vi "Index Tags.vi"(4 "Don't Create":bool, 6 "Tag Type":T1, 8 "error in (no error)":errorcluster, 9 "Tag":string, 10 "Group Index":i32, 11 "bt_Blackboard in":refnum<class "Blackboard.lvclass">) -> (0 "error out":errorcluster, 1 "New Tag?":bool, 2 "Value":refnum<class "Abs_Value.lvclass">, 3 "bt_Blackboard out":refnum<class "Blackboard.lvclass">)   [LabVIEW 2021, in "Blackboard.lvclass"]
uses:
  Blackboard.lvclass
  <vilib>/Utility/Data Type/Type Definitions/Data Type.ctl
  <vilib>/TSA/Abstract Data Classes/Abs_Types/Value/Abs_Value.lvclass
  Blackboard.lvclass/Blackboard.ctl
  <vilib>/TSA/Omni-Bus/Local Bus/Support/DBL/Local Bus_DBL.lvclass
  C:/Program Files (x86)/National Instruments/LabVIEW 2021/vi.lib/TSA/Abstract Data Classes/Abs_Types/Value/Abs_Value.lvclass
  <vilib>/TSA/Omni-Bus/Local Bus/Support/SGL/Local Bus_SGL.lvclass
  <vilib>/TSA/Omni-Bus/Local Bus/Support/EXT/Local Bus_EXT.lvclass
  <vilib>/TSA/Omni-Bus/Local Bus/Support/Bool/Local Bus_Boolean.lvclass
  <vilib>/TSA/Omni-Bus/Local Bus/Support/STR/Local Bus_String.lvclass
  <vilib>/TSA/Omni-Bus/Local Bus/Support/Variant/Local Bus_Variant.lvclass
  <vilib>/TSA/Omni-Bus/Local Bus/Support/WFM/Local Bus_Waveform.lvclass
  <vilib>/TSA/Omni-Bus/Local Bus/Support/Time/Local Bus_Time.lvclass
  <vilib>/TSA/Omni-Bus/Local Bus/Support/U8/Local Bus_U8.lvclass
  <vilib>/TSA/Omni-Bus/Local Bus/Support/U16/Local Bus_U16.lvclass
  <vilib>/TSA/Omni-Bus/Local Bus/Support/U32/Local Bus_U32.lvclass
  <vilib>/TSA/Omni-Bus/Local Bus/Support/U64/Local Bus_U64.lvclass
  <vilib>/TSA/Omni-Bus/Local Bus/Support/I8/Local Bus_I8.lvclass
  <vilib>/TSA/Omni-Bus/Local Bus/Support/I16/Local Bus_I16.lvclass
  <vilib>/TSA/Omni-Bus/Local Bus/Support/I32/Local Bus_I32.lvclass
  <vilib>/TSA/Omni-Bus/Local Bus/Support/I64/Local Bus_I64.lvclass
  <vilib>/TSA/Omni-Bus/Local Bus/Support/CSGL/Local Bus_CSGL.lvclass
  <vilib>/TSA/Omni-Bus/Local Bus/Support/CDBL/Local Bus_CDBL.lvclass
  <vilib>/TSA/Omni-Bus/Local Bus/Support/CEXT/Local Bus_CEXT.lvclass
  <vilib>/TSA/Omni-Bus/Local Bus/Support/Type/Local Bus_Type.lvclass
  <vilib>/TSA/Abstract Data Classes/Abs_Types/Type/Abs_Type.lvclass
  C:/Program Files (x86)/National Instruments/LabVIEW 2021/vi.lib/TSA/Abstract Data Classes/Abs_Types/Type/Abs_Type.lvclass
  C:/Program Files (x86)/National Instruments/LabVIEW 2021/vi.lib/TSA/Abstract Data Classes/Abs_Types/Double Float/Abs_Double Float.lvclass
  C:/Program Files (x86)/National Instruments/LabVIEW 2021/vi.lib/TSA/Abstract Data Classes/Abs_Types/Floating Point/Abs_Floating Point.lvclass
  C:/Program Files (x86)/National Instruments/LabVIEW 2021/vi.lib/TSA/Abstract Data Classes/Abs_Types/Numeric/Abs_Numeric.lvclass
  C:/Program Files (x86)/National Instruments/LabVIEW 2021/vi.lib/TSA/Omni-Bus/Local Bus/Support/DBL/Local Bus_DBL.lvclass
  C:/Program Files (x86)/National Instruments/LabVIEW 2021/vi.lib/TSA/Omni-Bus/Local Bus/Support/Interface/Local Bus_Int.lvclass
  C:/Program Files (x86)/National Instruments/LabVIEW 2021/vi.lib/TSA/Abstract Data Classes/Abs_Types/Single Float/Abs_Single Float.lvclass
  C:/Program Files (x86)/National Instruments/LabVIEW 2021/vi.lib/TSA/Omni-Bus/Local Bus/Support/SGL/Local Bus_SGL.lvclass
  C:/Program Files (x86)/National Instruments/LabVIEW 2021/vi.lib/TSA/Abstract Data Classes/Abs_Types/Extended Float/Abs_Extended Float.lvclass
  C:/Program Files (x86)/National Instruments/LabVIEW 2021/vi.lib/TSA/Omni-Bus/Local Bus/Support/EXT/Local Bus_EXT.lvclass
  C:/Program Files (x86)/National Instruments/LabVIEW 2021/vi.lib/TSA/Abstract Data Classes/Abs_Types/Boolean/Abs_Boolean.lvclass
  C:/Program Files (x86)/National Instruments/LabVIEW 2021/vi.lib/TSA/Omni-Bus/Local Bus/Support/Bool/Local Bus_Boolean.lvclass
  C:/Program Files (x86)/National Instruments/LabVIEW 2021/vi.lib/TSA/Abstract Data Classes/Abs_Types/String/Abs_String.lvclass
  C:/Program Files (x86)/National Instruments/LabVIEW 2021/vi.lib/TSA/Omni-Bus/Local Bus/Support/STR/Local Bus_String.lvclass
  C:/Program Files (x86)/National Instruments/LabVIEW 2021/vi.lib/TSA/Abstract Data Classes/Abs_Types/Variant/Abs_Variant.lvclass
  C:/Program Files (x86)/National Instruments/LabVIEW 2021/vi.lib/TSA/Omni-Bus/Local Bus/Support/Variant/Local Bus_Variant.lvclass
  C:/Program Files (x86)/National Instruments/LabVIEW 2021/vi.lib/TSA/Abstract Data Classes/Abs_Types/Waveform/Abs_Waveform.lvclass
  C:/Program Files (x86)/National Instruments/LabVIEW 2021/vi.lib/TSA/Abstract Data Classes/Abs_Types/Collections/Vectors/Vector/Vector.lvclass
  C:/Program Files (x86)/National Instruments/LabVIEW 2021/vi.lib/TSA/Abstract Data Classes/Abs_Types/Iterator/Iterator.lvclass
  C:/Program Files (x86)/National Instruments/LabVIEW 2021/vi.lib/TSA/Abstract Data Classes/Abs_Types/Collections/Vectors/Vector_DBL/Vector_DBL.lvclass
  C:/Program Files (x86)/National Instruments/LabVIEW 2021/vi.lib/TSA/Omni-Bus/Local Bus/Support/WFM/Local Bus_Waveform.lvclass
  C:/Program Files (x86)/National Instruments/LabVIEW 2021/vi.lib/TSA/Abstract Data Classes/Abs_Types/Time/Abs_Time.lvclass
  C:/Program Files (x86)/National Instruments/LabVIEW 2021/vi.lib/TSA/Omni-Bus/Local Bus/Support/Time/Local Bus_Time.lvclass
  C:/Program Files (x86)/National Instruments/LabVIEW 2021/vi.lib/TSA/Abstract Data Classes/Abs_Types/U8 Integer/Abs_U8 Integer.lvclass
  C:/Program Files (x86)/National Instruments/LabVIEW 2021/vi.lib/TSA/Abstract Data Classes/Abs_Types/Integer/Abs_Integer.lvclass
  C:/Program Files (x86)/National Instruments/LabVIEW 2021/vi.lib/TSA/Omni-Bus/Local Bus/Support/U8/Local Bus_U8.lvclass
  C:/Program Files (x86)/National Instruments/LabVIEW 2021/vi.lib/TSA/Abstract Data Classes/Abs_Types/U16 Integer/Abs_U16 Integer.lvclass
  C:/Program Files (x86)/National Instruments/LabVIEW 2021/vi.lib/TSA/Omni-Bus/Local Bus/Support/U16/Local Bus_U16.lvclass
  C:/Program Files (x86)/National Instruments/LabVIEW 2021/vi.lib/TSA/Abstract Data Classes/Abs_Types/U32 Integer/Abs_U32 Integer.lvclass
  C:/Program Files (x86)/National Instruments/LabVIEW 2021/vi.lib/TSA/Omni-Bus/Local Bus/Support/U32/Local Bus_U32.lvclass
  C:/Program Files (x86)/National Instruments/LabVIEW 2021/vi.lib/TSA/Abstract Data Classes/Abs_Types/U64 Integer/Abs_U64 Integer.lvclass
  C:/Program Files (x86)/National Instruments/LabVIEW 2021/vi.lib/TSA/Omni-Bus/Local Bus/Support/U64/Local Bus_U64.lvclass
  C:/Program Files (x86)/National Instruments/LabVIEW 2021/vi.lib/TSA/Abstract Data Classes/Abs_Types/I8 Integer/Abs_I8 Integer.lvclass
  C:/Program Files (x86)/National Instruments/LabVIEW 2021/vi.lib/TSA/Omni-Bus/Local Bus/Support/I8/Local Bus_I8.lvclass
  C:/Program Files (x86)/National Instruments/LabVIEW 2021/vi.lib/TSA/Abstract Data Classes/Abs_Types/I16 Integer/Abs_I16 Integer.lvclass
  C:/Program Files (x86)/National Instruments/LabVIEW 2021/vi.lib/TSA/Omni-Bus/Local Bus/Support/I16/Local Bus_I16.lvclass
  C:/Program Files (x86)/National Instruments/LabVIEW 2021/vi.lib/TSA/Abstract Data Classes/Abs_Types/I32 Integer/Abs_I32 Integer.lvclass
  C:/Program Files (x86)/National Instruments/LabVIEW 2021/vi.lib/TSA/Omni-Bus/Local Bus/Support/I32/Local Bus_I32.lvclass
  C:/Program Files (x86)/National Instruments/LabVIEW 2021/vi.lib/TSA/Abstract Data Classes/Abs_Types/I64 Integer/Abs_I64 Integer.lvclass
  C:/Program Files (x86)/National Instruments/LabVIEW 2021/vi.lib/TSA/Omni-Bus/Local Bus/Support/I64/Local Bus_I64.lvclass
  C:/Program Files (x86)/National Instruments/LabVIEW 2021/vi.lib/TSA/Abstract Data Classes/Abs_Types/Complex Single Float/Abs_Complex Single Float.lvclass
  C:/Program Files (x86)/National Instruments/LabVIEW 2021/vi.lib/TSA/Omni-Bus/Local Bus/Support/CSGL/Local Bus_CSGL.lvclass
  C:/Program Files (x86)/National Instruments/LabVIEW 2021/vi.lib/TSA/Abstract Data Classes/Abs_Types/Complex Double Float/Abs_Complex Double Float.lvclass
  C:/Program Files (x86)/National Instruments/LabVIEW 2021/vi.lib/TSA/Omni-Bus/Local Bus/Support/CDBL/Local Bus_CDBL.lvclass
  C:/Program Files (x86)/National Instruments/LabVIEW 2021/vi.lib/TSA/Abstract Data Classes/Abs_Types/Complex Extended Float/Abs_Complex Extended Float.lvclass
  C:/Program Files (x86)/National Instruments/LabVIEW 2021/vi.lib/TSA/Omni-Bus/Local Bus/Support/CEXT/Local Bus_CEXT.lvclass
  <vilib>/Utility/Data Type/NI_Data Type.lvlib
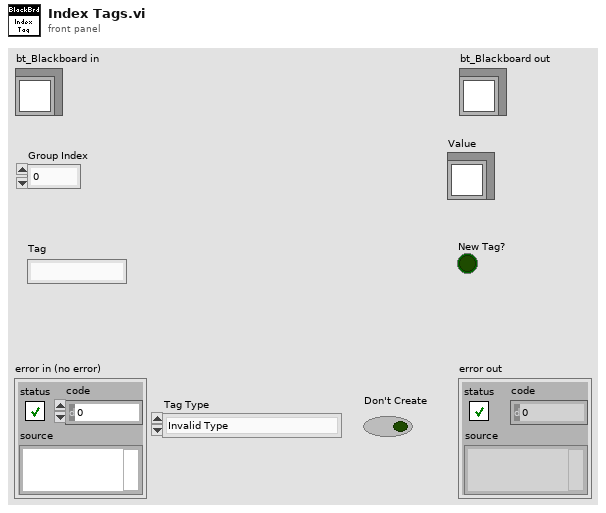
[diagram p1: front panel]
types:
  T1 = typedef "NI_Data Type.lvlib/Data Type.ctl" = enum8{"Invalid Type", "Void", "I8", "I16", "I32", "I64", "U8", "U16", "U32", "U64", "Single Float", "Double Float", "Extended Float", "Single Complex", "Double Complex", "Extended Complex", "Enum U8", "Enum U16", "Enum U32", "Enum U64", "Single Float With Unit", "Double Float With Unit", "Extended Float With Unit", "Single Complex with Unit", "Double Complex with Unit", "Extended Complex with Unit", "Boolean", "String", "Path", "Picture", "Tag", "Array", "Cluster", "Variant", "LV Variant", "Waveform", "Timestamp", "Digital Waveform", "Digital Data", "ExpressData", "Refnum", "External Data", "VI", "Poly VI", "LabVIEW Class Instance", "Fixed Point", "Set Collection", "Map Collection"}
  T2 = typedef "Blackboard.lvclass/Groups Type.ctl" = cluster{"Data":T3[], "Map":T6}
  T3 = typedef "Blackboard.lvclass/Data DVR Type.ctl" = cluster{"Tags":T4, "Data Refs":T5}
  T4 = typedef "Blackboard.lvclass/Tags Map Type.ctl" = map{string, refnum<class "Abs_Value.lvclass">}
  T5 = typedef "Local Bus.lvclass/Data Value References.ctl" = cluster{"Boolean":refnum<data-value>, "String":refnum<data-value>, "DBL":refnum<data-value>, "SGL":refnum<data-value>, "EXT":refnum<data-value>, "U8":refnum<data-value>, "U16":refnum<data-value>, "U32":refnum<data-value>, "U64":refnum<data-value>, "I8":refnum<data-value>, "I16":refnum<data-value>, "I32":refnum<data-value>, "I64":refnum<data-value>, "CDBL":refnum<data-value>, "CSGL":refnum<data-value>, "CEXT":refnum<data-value>, "Time":refnum<data-value>, "Variant":refnum<data-value>, "Waveform":refnum<data-value>, "Type":refnum<data-value>}
  T6 = typedef "Blackboard.lvclass/Group Map Type.ctl" = map{string, i32}
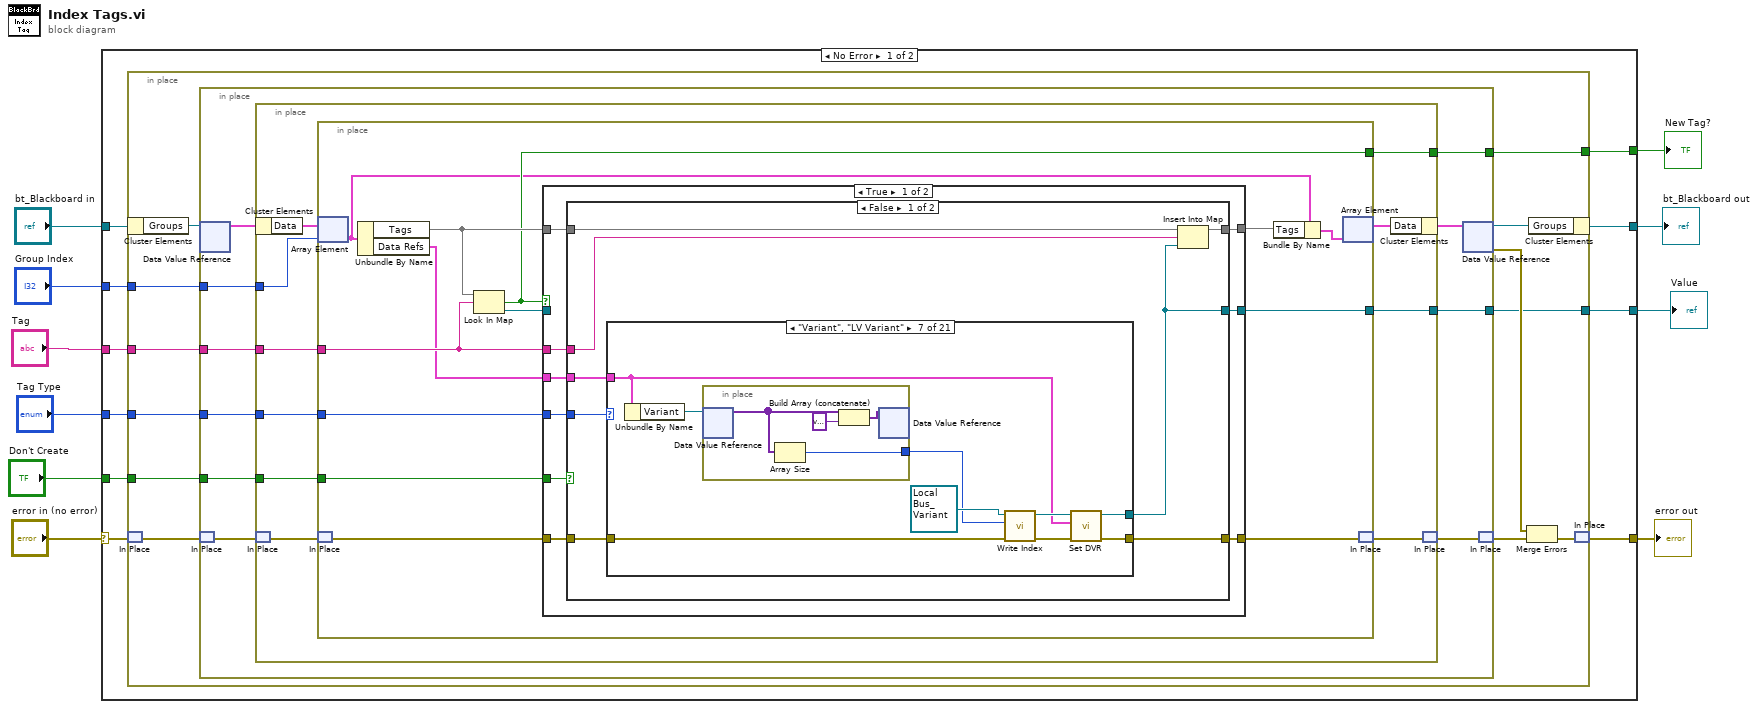
[diagram p0: block diagram]
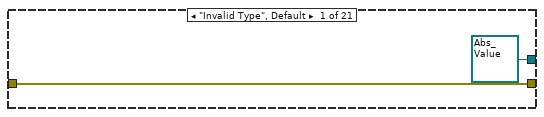
[diagram p2: hidden frame]
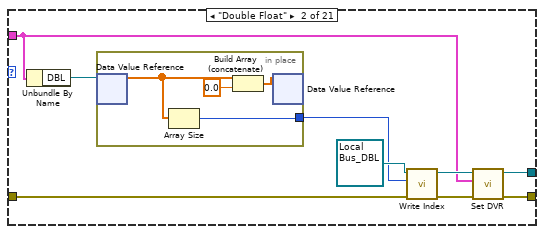
[diagram p3: hidden frame]
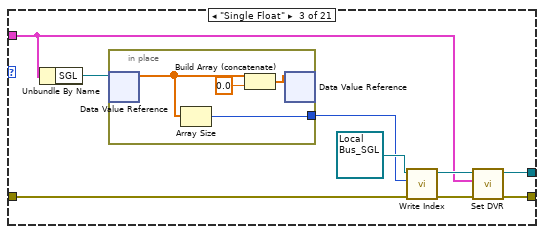
[diagram p4: hidden frame]
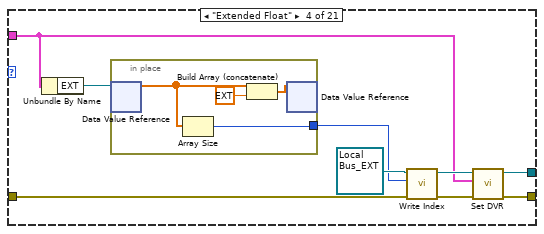
[diagram p5: hidden frame]
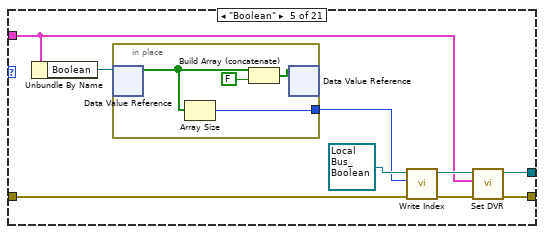
[diagram p6: hidden frame]
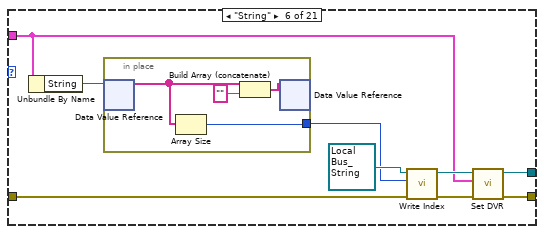
[diagram p7: hidden frame]
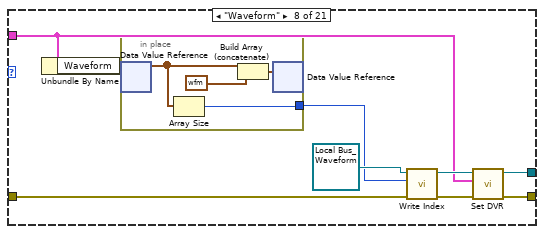
[diagram p8: hidden frame]
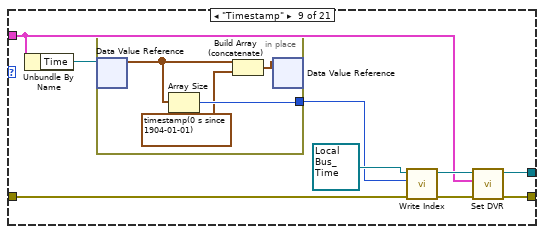
[diagram p9: hidden frame]
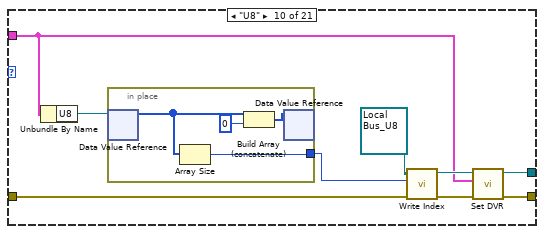
[diagram p10: hidden frame]
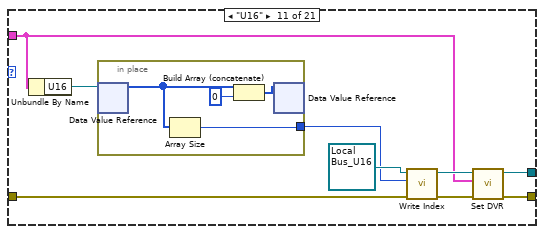
[diagram p11: hidden frame]
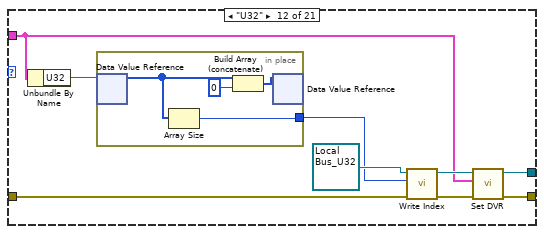
[diagram p12: hidden frame]
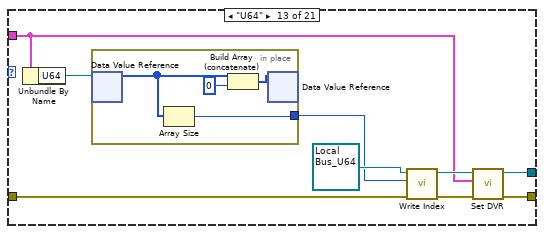
[diagram p13: hidden frame]
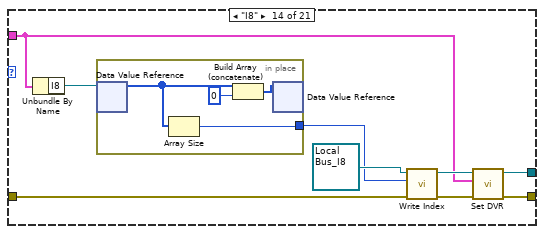
[diagram p14: hidden frame]
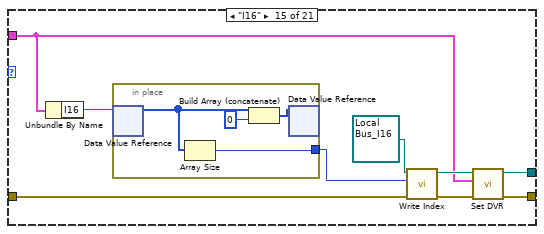
[diagram p15: hidden frame]
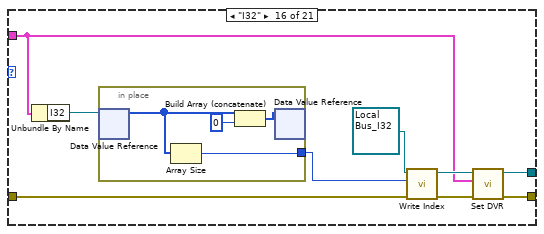
[diagram p16: hidden frame]
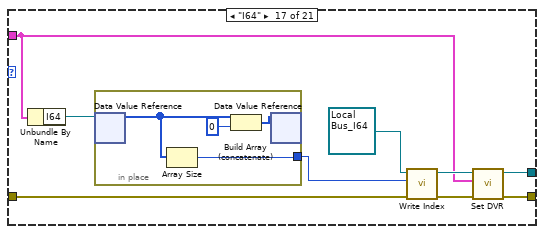
[diagram p17: hidden frame]
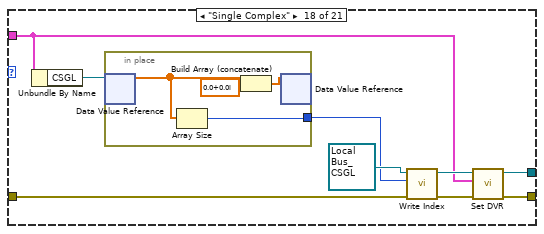
[diagram p18: hidden frame]
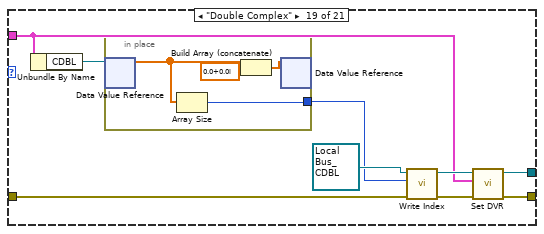
[diagram p19: hidden frame]
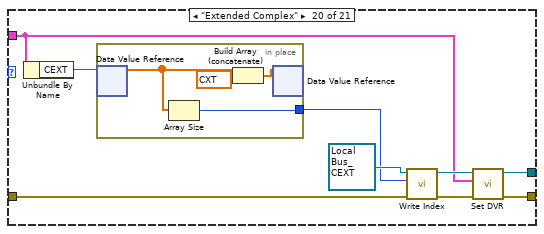
[diagram p20: hidden frame]
diagram:
  n1 = case shown="No Error" "error in (no error)" {
    selector: "error in (no error)" -> [w16 w355]
    tunnel: [w15 w355] -> w9
    tunnel: [w18 w354] -> w7
    tunnel: "bt_Blackboard in" -> [w19 w354]
    tunnel: "Tag" -> [w20 _]
    tunnel: "Group Index" -> [w17 _]
    tunnel: [w14 _] -> w4
    tunnel: [w13 _] -> w2
    tunnel: "Tag Type" -> [w12 _]
    tunnel: "Don't Create" -> [w11 _]
    frame No Error {
      n2 = in-place {
        in-place-border: w20 -> [w32]
        in-place-border: w17 -> [w31]
        in-place-border: [w30] -> w14
        in-place-border: [w23] -> w13
        in-place-border: w12 -> [w22]
        in-place-border: w11 -> [w21]
        n3 = in-place-cluster #1(w19) -> ("Groups"=w29:refnum<data-value>)
        n4 = in-place-match #2(w16) -> (w28:errorcluster)
        n5 = in-place {
          in-place-border: w32 -> [w42]
          in-place-border: w31 -> [w41]
          in-place-border: [w40] -> w30
          in-place-border: [w35] -> w23
          in-place-border: w22 -> [w34]
          in-place-border: w21 -> [w33]
          n6 = in-place-dvr #3(w29) -> (w39:T2)  [unwired: 1 out]
          n7 = in-place-match #4(w28) -> (w37:errorcluster)
          n8 = in-place {
            in-place-border: w42 -> [w52]
            in-place-border: w41 -> [w51]
            in-place-border: [w50] -> w40
            in-place-border: [w45] -> w35
            in-place-border: w34 -> [w44]
            in-place-border: w33 -> [w43]
            n9 = in-place-cluster #5(w39) -> ("Data"=w49:T3[])
            n10 = in-place-match #6(w37) -> (w47:errorcluster)
            n11 = in-place {
              in-place-border: w52 -> [w57]
              in-place-border: [w60] -> w50
              in-place-border: [w59] -> w45
              in-place-border: w44 -> [w55]
              in-place-border: w43 -> [w53]
              n12 = in-place-array #7(w49, w51) -> (w54:T3)
              n13 = in-place-match #8(w47) -> (w65:errorcluster)
              n14 = Unbundle By Name(w54) -> ("Tags"=w63:T4, "Data Refs"=w56:T5)
              n15 = Look In Map(map=w63, key=w57) -> (key not found?=w60:bool, value=w61:refnum<class "Abs_Value.lvclass">)  [unwired: 1 in]
              n16 = case shown="True" w60 {
                tunnel: w63 -> [w74 w353]
                tunnel: [w73 w353] -> w62
                tunnel: w65 -> [w70 w352]
                tunnel: [w69 w352] -> w64
                tunnel: w61 -> [_ w351]
                tunnel: [w67 w351] -> w59
                tunnel: w57 -> [w72 _]
                tunnel: w56 -> [w71 _]
                tunnel: w55 -> [w68 _]
                tunnel: w53 -> [w66 _]
                frame True {
                  n17 = case shown="False" w66 {
                    tunnel: w74 -> [w82 w350]
                    tunnel: [w81 w350] -> w73
                    tunnel: w72 -> [w80 _]
                    tunnel: w71 -> [w79 _]
                    tunnel: w70 -> [w78 w348]
                    tunnel: [w77 w348] -> w69
                    tunnel: w68 -> [w76 _]
                    tunnel: [w75 refnum<class "Abs_Value.lvclass"> refnum ("Local Bus_DBL out")] -> w67
                    frame False {
                      n18 = case shown="\"Variant\", \"LV Variant\"" w76 {
                        tunnel: [w84 w93 w106 w119 w132 w145 w158 w171 w184 w197 w210 w223 w236 w249 w262 w275 w288 w301 w314 w327 w336] -> w77
                        tunnel: w79 -> [_ w86 w99 w112 w125 w138 w151 w164 w177 w190 w203 w216 w229 w242 w255 w268 w281 w294 w307 w320 w339]
                        tunnel: [refnum<class "Abs_Value.lvclass"> refnum ("Local Bus_DBL out") w92 w105 w118 w131 w144 w157 w170 w183 w196 w209 w222 w235 w248 w261 w274 w287 w300 w313 w326 w332] -> w75
                        tunnel: w78 -> [w84 w91 w104 w117 w130 w143 w156 w169 w182 w195 w208 w221 w234 w247 w260 w273 w286 w299 w312 w325 w343]
                        frame "Invalid Type", Default {
                        }
                        frame "Double Float" {
                          n19 = Unbundle By Name(w86) -> ("DBL"=w87:refnum<data-value>)
                          n20 = in-place {
                            in-place-border: [w95] -> w85
                            n21 = in-place-dvr #9(w87) -> (w96:dbl[])  [unwired: 1 out]
                            n22 = Array Size(array=w96) -> (size(s)=w95:i32)
                            n23 = Build Array (concatenate)(w96, 0.0 ("element")) -> (w97:dbl[])
                            n24 = in-place-dvr #9(w97) -> ()  [unwired: 2 out]
                          }
                          n25 = call-dynamic "Write Index.vi"("error in (no error)"=w91, "Index"=w85, "Local Bus_Access in"=refnum<class "Local Bus_DBL.lvclass"> refnum ("Local Bus_DBL.lvclass")) -> ("error out"=w90:errorcluster, "Local Bus_Access out"=w89:refnum<class "Local Bus_DBL.lvclass">)  [unwired: 7 in]
                          n26 = call-dynamic "Set DVR.vi"("error in (no error)"=w90, "Type Counts"=w86, "Local Bus_DBL in"=w89) -> ("error out"=w93:errorcluster, "Local Bus_DBL out"=w92:refnum<class "Local Bus_DBL.lvclass">)  [unwired: 7 in]
                        }
                        frame "Single Float" {
                          n27 = Unbundle By Name(w99) -> ("SGL"=w100:refnum<data-value>)
                          n28 = in-place {
                            in-place-border: [w108] -> w98
                            n29 = in-place-dvr #10(w100) -> (w109:sgl[])  [unwired: 1 out]
                            n30 = Array Size(array=w109) -> (size(s)=w108:i32)
                            n31 = Build Array (concatenate)(w109, sgl 0.0 ("element")) -> (w110:sgl[])
                            n32 = in-place-dvr #10(w110) -> ()  [unwired: 2 out]
                          }
                          n33 = call-dynamic "Write Index.vi"("error in (no error)"=w104, "Index"=w98, "Local Bus_Access in"=refnum<class "Local Bus_SGL.lvclass"> refnum ("Local Bus_SGL.lvclass")) -> ("error out"=w103:errorcluster, "Local Bus_Access out"=w102:refnum<class "Local Bus_SGL.lvclass">)  [unwired: 7 in]
                          n34 = call-dynamic "Set DVR.vi"("error in (no error)"=w103, "Type Counts"=w99, "Local Bus_DBL in"=w102) -> ("error out"=w106:errorcluster, "Local Bus_DBL out"=w105:refnum<class "Local Bus_SGL.lvclass">)  [unwired: 7 in]
                        }
                        frame "Extended Float" {
                          n35 = Unbundle By Name(w112) -> ("EXT"=w113:refnum<data-value>)
                          n36 = in-place {
                            in-place-border: [w121] -> w111
                            n37 = in-place-dvr #11(w113) -> (w122:ext[])  [unwired: 1 out]
                            n38 = Array Size(array=w122) -> (size(s)=w121:i32)
                            n39 = Build Array (concatenate)(w122, ext 0.0 ("element")) -> (w123:ext[])
                            n40 = in-place-dvr #11(w123) -> ()  [unwired: 2 out]
                          }
                          n41 = call-dynamic "Write Index.vi"("error in (no error)"=w117, "Index"=w111, "Local Bus_Access in"=refnum<class "Local Bus_EXT.lvclass"> refnum ("Local Bus_EXT.lvclass")) -> ("error out"=w116:errorcluster, "Local Bus_Access out"=w115:refnum<class "Local Bus_EXT.lvclass">)  [unwired: 7 in]
                          n42 = call-dynamic "Set DVR.vi"("error in (no error)"=w116, "Type Counts"=w112, "Local Bus_DBL in"=w115) -> ("error out"=w119:errorcluster, "Local Bus_DBL out"=w118:refnum<class "Local Bus_EXT.lvclass">)  [unwired: 7 in]
                        }
                        frame "Boolean" {
                          n43 = Unbundle By Name(w125) -> ("Boolean"=w126:refnum<data-value>)
                          n44 = in-place {
                            in-place-border: [w134] -> w124
                            n45 = in-place-dvr #12(w126) -> (w135:bool[])  [unwired: 1 out]
                            n46 = Array Size(array=w135) -> (size(s)=w134:i32)
                            n47 = Build Array (concatenate)(w135, FALSE ("Boolean")) -> (w136:bool[])
                            n48 = in-place-dvr #12(w136) -> ()  [unwired: 2 out]
                          }
                          n49 = call-dynamic "Write Index.vi"("error in (no error)"=w130, "Index"=w124, "Local Bus_Access in"=refnum<class "Local Bus_Boolean.lvclass"> refnum ("Local Bus_Boolean.lvclass")) -> ("error out"=w129:errorcluster, "Local Bus_Access out"=w128:refnum<class "Local Bus_Boolean.lvclass">)  [unwired: 7 in]
                          n50 = call-dynamic "Set DVR.vi"("error in (no error)"=w129, "Type Counts"=w125, "Local Bus_DBL in"=w128) -> ("error out"=w132:errorcluster, "Local Bus_DBL out"=w131:refnum<class "Local Bus_Boolean.lvclass">)  [unwired: 7 in]
                        }
                        frame "String" {
                          n51 = Unbundle By Name(w138) -> ("String"=w139:refnum<data-value>)
                          n52 = in-place {
                            in-place-border: [w147] -> w137
                            n53 = in-place-dvr #13(w139) -> (w148:string[])  [unwired: 1 out]
                            n54 = Array Size(array=w148) -> (size(s)=w147:i32)
                            n55 = Build Array (concatenate)(w148, "" ("element")) -> (w149:string[])
                            n56 = in-place-dvr #13(w149) -> ()  [unwired: 2 out]
                          }
                          n57 = call-dynamic "Write Index.vi"("error in (no error)"=w143, "Index"=w137, "Local Bus_Access in"=refnum<class "Local Bus_String.lvclass"> refnum ("Local Bus_String.lvclass")) -> ("error out"=w142:errorcluster, "Local Bus_Access out"=w141:refnum<class "Local Bus_String.lvclass">)  [unwired: 7 in]
                          n58 = call-dynamic "Set DVR.vi"("error in (no error)"=w142, "Type Counts"=w138, "Local Bus_DBL in"=w141) -> ("error out"=w145:errorcluster, "Local Bus_DBL out"=w144:refnum<class "Local Bus_String.lvclass">)  [unwired: 7 in]
                        }
                        frame "Variant", "LV Variant" {
                          n59 = Unbundle By Name(w151) -> ("Variant"=w152:refnum<data-value>)
                          n60 = in-place {
                            in-place-border: [w160] -> w150
                            n61 = in-place-dvr #14(w152) -> (w161:variant[])  [unwired: 1 out]
                            n62 = Array Size(array=w161) -> (size(s)=w160:i32)
                            n63 = Build Array (concatenate)(w161, variant ("element")) -> (w162:variant[])
                            n64 = in-place-dvr #14(w162) -> ()  [unwired: 2 out]
                          }
                          n65 = call-dynamic "Write Index.vi"("error in (no error)"=w156, "Index"=w150, "Local Bus_Access in"=refnum<class "Local Bus_Variant.lvclass"> refnum ("Local Bus_Variant.lvclass")) -> ("error out"=w155:errorcluster, "Local Bus_Access out"=w154:refnum<class "Local Bus_Variant.lvclass">)  [unwired: 7 in]
                          n66 = call-dynamic "Set DVR.vi"("error in (no error)"=w155, "Type Counts"=w151, "Local Bus_DBL in"=w154) -> ("error out"=w158:errorcluster, "Local Bus_DBL out"=w157:refnum<class "Local Bus_Variant.lvclass">)  [unwired: 7 in]
                        }
                        frame "Waveform" {
                          n67 = Unbundle By Name(w164) -> ("Waveform"=w165:refnum<data-value>)
                          n68 = in-place {
                            in-place-border: [w173] -> w163
                            n69 = in-place-dvr #15(w165) -> (w174:waveform(dbl)[])  [unwired: 1 out]
                            n70 = Array Size(array=w174) -> (size(s)=w173:i32)
                            n71 = Build Array (concatenate)(w174, waveform(dbl) {"t0"=timestamp(0 s since 1904-01-01), "dt"=1.0, "Y"=[]} ("element")) -> (w175:waveform(dbl)[])
                            n72 = in-place-dvr #15(w175) -> ()  [unwired: 2 out]
                          }
                          n73 = call-dynamic "Write Index.vi"("error in (no error)"=w169, "Index"=w163, "Local Bus_Access in"=refnum<class "Local Bus_Waveform.lvclass"> refnum ("Local Bus_Waveform.lvclass")) -> ("error out"=w168:errorcluster, "Local Bus_Access out"=w167:refnum<class "Local Bus_Waveform.lvclass">)  [unwired: 7 in]
                          n74 = call-dynamic "Set DVR.vi"("error in (no error)"=w168, "Type Counts"=w164, "Local Bus_DBL in"=w167) -> ("error out"=w171:errorcluster, "Local Bus_DBL out"=w170:refnum<class "Local Bus_Waveform.lvclass">)  [unwired: 7 in]
                        }
                        frame "Timestamp" {
                          n75 = Unbundle By Name(w177) -> ("Time"=w178:refnum<data-value>)
                          n76 = in-place {
                            in-place-border: [w186] -> w176
                            n77 = in-place-dvr #16(w178) -> (w187:timestamp[])  [unwired: 1 out]
                            n78 = Array Size(array=w187) -> (size(s)=w186:i32)
                            n79 = Build Array (concatenate)(w187, timestamp(0 s since 1904-01-01) ("element")) -> (w188:timestamp[])
                            n80 = in-place-dvr #16(w188) -> ()  [unwired: 2 out]
                          }
                          n81 = call-dynamic "Write Index.vi"("error in (no error)"=w182, "Index"=w176, "Local Bus_Access in"=refnum<class "Local Bus_Time.lvclass"> refnum ("Local Bus_Time.lvclass")) -> ("error out"=w181:errorcluster, "Local Bus_Access out"=w180:refnum<class "Local Bus_Time.lvclass">)  [unwired: 7 in]
                          n82 = call-dynamic "Set DVR.vi"("error in (no error)"=w181, "Type Counts"=w177, "Local Bus_DBL in"=w180) -> ("error out"=w184:errorcluster, "Local Bus_DBL out"=w183:refnum<class "Local Bus_Time.lvclass">)  [unwired: 7 in]
                        }
                        frame "U8" {
                          n83 = Unbundle By Name(w190) -> ("U8"=w191:refnum<data-value>)
                          n84 = in-place {
                            in-place-border: [w199] -> w189
                            n85 = in-place-dvr #17(w191) -> (w200:u8[])  [unwired: 1 out]
                            n86 = Array Size(array=w200) -> (size(s)=w199:i32)
                            n87 = Build Array (concatenate)(w200, u8 0 ("element")) -> (w201:u8[])
                            n88 = in-place-dvr #17(w201) -> ()  [unwired: 2 out]
                          }
                          n89 = call-dynamic "Write Index.vi"("error in (no error)"=w195, "Index"=w189, "Local Bus_Access in"=refnum<class "Local Bus_U8.lvclass"> refnum ("Local Bus_U8.lvclass")) -> ("error out"=w194:errorcluster, "Local Bus_Access out"=w193:refnum<class "Local Bus_U8.lvclass">)  [unwired: 7 in]
                          n90 = call-dynamic "Set DVR.vi"("error in (no error)"=w194, "Type Counts"=w190, "Local Bus_DBL in"=w193) -> ("error out"=w197:errorcluster, "Local Bus_DBL out"=w196:refnum<class "Local Bus_U8.lvclass">)  [unwired: 7 in]
                        }
                        frame "U16" {
                          n91 = Unbundle By Name(w203) -> ("U16"=w204:refnum<data-value>)
                          n92 = in-place {
                            in-place-border: [w212] -> w202
                            n93 = in-place-dvr #18(w204) -> (w213:u16[])  [unwired: 1 out]
                            n94 = Array Size(array=w213) -> (size(s)=w212:i32)
                            n95 = Build Array (concatenate)(w213, u16 0 ("element")) -> (w214:u16[])
                            n96 = in-place-dvr #18(w214) -> ()  [unwired: 2 out]
                          }
                          n97 = call-dynamic "Write Index.vi"("error in (no error)"=w208, "Index"=w202, "Local Bus_Access in"=refnum<class "Local Bus_U16.lvclass"> refnum ("Local Bus_U16.lvclass")) -> ("error out"=w207:errorcluster, "Local Bus_Access out"=w206:refnum<class "Local Bus_U16.lvclass">)  [unwired: 7 in]
                          n98 = call-dynamic "Set DVR.vi"("error in (no error)"=w207, "Type Counts"=w203, "Local Bus_DBL in"=w206) -> ("error out"=w210:errorcluster, "Local Bus_DBL out"=w209:refnum<class "Local Bus_U16.lvclass">)  [unwired: 7 in]
                        }
                        frame "U32" {
                          n99 = Unbundle By Name(w216) -> ("U32"=w217:refnum<data-value>)
                          n100 = in-place {
                            in-place-border: [w225] -> w215
                            n101 = in-place-dvr #19(w217) -> (w226:u32[])  [unwired: 1 out]
                            n102 = Array Size(array=w226) -> (size(s)=w225:i32)
                            n103 = Build Array (concatenate)(w226, u32 0 ("element")) -> (w227:u32[])
                            n104 = in-place-dvr #19(w227) -> ()  [unwired: 2 out]
                          }
                          n105 = call-dynamic "Write Index.vi"("error in (no error)"=w221, "Index"=w215, "Local Bus_Access in"=refnum<class "Local Bus_U32.lvclass"> refnum ("Local Bus_U32.lvclass")) -> ("error out"=w220:errorcluster, "Local Bus_Access out"=w219:refnum<class "Local Bus_U32.lvclass">)  [unwired: 7 in]
                          n106 = call-dynamic "Set DVR.vi"("error in (no error)"=w220, "Type Counts"=w216, "Local Bus_DBL in"=w219) -> ("error out"=w223:errorcluster, "Local Bus_DBL out"=w222:refnum<class "Local Bus_U32.lvclass">)  [unwired: 7 in]
                        }
                        frame "U64" {
                          n107 = Unbundle By Name(w229) -> ("U64"=w230:refnum<data-value>)
                          n108 = in-place {
                            in-place-border: [w238] -> w228
                            n109 = in-place-dvr #20(w230) -> (w239:u64[])  [unwired: 1 out]
                            n110 = Array Size(array=w239) -> (size(s)=w238:i32)
                            n111 = Build Array (concatenate)(w239, u64 0 ("element")) -> (w240:u64[])
                            n112 = in-place-dvr #20(w240) -> ()  [unwired: 2 out]
                          }
                          n113 = call-dynamic "Write Index.vi"("error in (no error)"=w234, "Index"=w228, "Local Bus_Access in"=refnum<class "Local Bus_U64.lvclass"> refnum ("Local Bus_U64.lvclass")) -> ("error out"=w233:errorcluster, "Local Bus_Access out"=w232:refnum<class "Local Bus_U64.lvclass">)  [unwired: 7 in]
                          n114 = call-dynamic "Set DVR.vi"("error in (no error)"=w233, "Type Counts"=w229, "Local Bus_DBL in"=w232) -> ("error out"=w236:errorcluster, "Local Bus_DBL out"=w235:refnum<class "Local Bus_U64.lvclass">)  [unwired: 7 in]
                        }
                        frame "I8" {
                          n115 = Unbundle By Name(w242) -> ("I8"=w243:refnum<data-value>)
                          n116 = in-place {
                            in-place-border: [w251] -> w241
                            n117 = in-place-dvr #21(w243) -> (w252:i8[])  [unwired: 1 out]
                            n118 = Array Size(array=w252) -> (size(s)=w251:i32)
                            n119 = Build Array (concatenate)(w252, i8 0 ("element")) -> (w253:i8[])
                            n120 = in-place-dvr #21(w253) -> ()  [unwired: 2 out]
                          }
                          n121 = call-dynamic "Write Index.vi"("error in (no error)"=w247, "Index"=w241, "Local Bus_Access in"=refnum<class "Local Bus_I8.lvclass"> refnum ("Local Bus_I8.lvclass")) -> ("error out"=w246:errorcluster, "Local Bus_Access out"=w245:refnum<class "Local Bus_I8.lvclass">)  [unwired: 7 in]
                          n122 = call-dynamic "Set DVR.vi"("error in (no error)"=w246, "Type Counts"=w242, "Local Bus_DBL in"=w245) -> ("error out"=w249:errorcluster, "Local Bus_DBL out"=w248:refnum<class "Local Bus_I8.lvclass">)  [unwired: 7 in]
                        }
                        frame "I16" {
                          n123 = Unbundle By Name(w255) -> ("I16"=w256:refnum<data-value>)
                          n124 = in-place {
                            in-place-border: [w264] -> w254
                            n125 = in-place-dvr #22(w256) -> (w265:i16[])  [unwired: 1 out]
                            n126 = Array Size(array=w265) -> (size(s)=w264:i32)
                            n127 = Build Array (concatenate)(w265, i16 0 ("element")) -> (w266:i16[])
                            n128 = in-place-dvr #22(w266) -> ()  [unwired: 2 out]
                          }
                          n129 = call-dynamic "Write Index.vi"("error in (no error)"=w260, "Index"=w254, "Local Bus_Access in"=refnum<class "Local Bus_I16.lvclass"> refnum ("Local Bus_I16.lvclass")) -> ("error out"=w259:errorcluster, "Local Bus_Access out"=w258:refnum<class "Local Bus_I16.lvclass">)  [unwired: 7 in]
                          n130 = call-dynamic "Set DVR.vi"("error in (no error)"=w259, "Type Counts"=w255, "Local Bus_DBL in"=w258) -> ("error out"=w262:errorcluster, "Local Bus_DBL out"=w261:refnum<class "Local Bus_I16.lvclass">)  [unwired: 7 in]
                        }
                        frame "I32" {
                          n131 = Unbundle By Name(w268) -> ("I32"=w269:refnum<data-value>)
                          n132 = in-place {
                            in-place-border: [w277] -> w267
                            n133 = in-place-dvr #23(w269) -> (w278:i32[])  [unwired: 1 out]
                            n134 = Array Size(array=w278) -> (size(s)=w277:i32)
                            n135 = Build Array (concatenate)(w278, 0 ("element")) -> (w279:i32[])
                            n136 = in-place-dvr #23(w279) -> ()  [unwired: 2 out]
                          }
                          n137 = call-dynamic "Write Index.vi"("error in (no error)"=w273, "Index"=w267, "Local Bus_Access in"=refnum<class "Local Bus_I32.lvclass"> refnum ("Local Bus_I32.lvclass")) -> ("error out"=w272:errorcluster, "Local Bus_Access out"=w271:refnum<class "Local Bus_I32.lvclass">)  [unwired: 7 in]
                          n138 = call-dynamic "Set DVR.vi"("error in (no error)"=w272, "Type Counts"=w268, "Local Bus_DBL in"=w271) -> ("error out"=w275:errorcluster, "Local Bus_DBL out"=w274:refnum<class "Local Bus_I32.lvclass">)  [unwired: 7 in]
                        }
                        frame "I64" {
                          n139 = Unbundle By Name(w281) -> ("I64"=w282:refnum<data-value>)
                          n140 = in-place {
                            in-place-border: [w290] -> w280
                            n141 = in-place-dvr #24(w282) -> (w291:i64[])  [unwired: 1 out]
                            n142 = Array Size(array=w291) -> (size(s)=w290:i32)
                            n143 = Build Array (concatenate)(w291, i64 0 ("element")) -> (w292:i64[])
                            n144 = in-place-dvr #24(w292) -> ()  [unwired: 2 out]
                          }
                          n145 = call-dynamic "Write Index.vi"("error in (no error)"=w286, "Index"=w280, "Local Bus_Access in"=refnum<class "Local Bus_I64.lvclass"> refnum ("Local Bus_I64.lvclass")) -> ("error out"=w285:errorcluster, "Local Bus_Access out"=w284:refnum<class "Local Bus_I64.lvclass">)  [unwired: 7 in]
                          n146 = call-dynamic "Set DVR.vi"("error in (no error)"=w285, "Type Counts"=w281, "Local Bus_DBL in"=w284) -> ("error out"=w288:errorcluster, "Local Bus_DBL out"=w287:refnum<class "Local Bus_I64.lvclass">)  [unwired: 7 in]
                        }
                        frame "Single Complex" {
                          n147 = Unbundle By Name(w294) -> ("CSGL"=w295:refnum<data-value>)
                          n148 = in-place {
                            in-place-border: [w303] -> w293
                            n149 = in-place-dvr #25(w295) -> (w304:csg[])  [unwired: 1 out]
                            n150 = Array Size(array=w304) -> (size(s)=w303:i32)
                            n151 = Build Array (concatenate)(w304, csg 0.0+0.0i ("element")) -> (w305:csg[])
                            n152 = in-place-dvr #25(w305) -> ()  [unwired: 2 out]
                          }
                          n153 = call-dynamic "Write Index.vi"("error in (no error)"=w299, "Index"=w293, "Local Bus_Access in"=refnum<class "Local Bus_CSGL.lvclass"> refnum ("Local Bus_CSGL.lvclass")) -> ("error out"=w298:errorcluster, "Local Bus_Access out"=w297:refnum<class "Local Bus_CSGL.lvclass">)  [unwired: 7 in]
                          n154 = call-dynamic "Set DVR.vi"("error in (no error)"=w298, "Type Counts"=w294, "Local Bus_DBL in"=w297) -> ("error out"=w301:errorcluster, "Local Bus_DBL out"=w300:refnum<class "Local Bus_CSGL.lvclass">)  [unwired: 7 in]
                        }
                        frame "Double Complex" {
                          n155 = Unbundle By Name(w307) -> ("CDBL"=w308:refnum<data-value>)
                          n156 = in-place {
                            in-place-border: [w316] -> w306
                            n157 = in-place-dvr #26(w308) -> (w317:cdb[])  [unwired: 1 out]
                            n158 = Array Size(array=w317) -> (size(s)=w316:i32)
                            n159 = Build Array (concatenate)(w317, cdb 0.0+0.0i ("element")) -> (w318:cdb[])
                            n160 = in-place-dvr #26(w318) -> ()  [unwired: 2 out]
                          }
                          n161 = call-dynamic "Write Index.vi"("error in (no error)"=w312, "Index"=w306, "Local Bus_Access in"=refnum<class "Local Bus_CDBL.lvclass"> refnum ("Local Bus_CDBL.lvclass")) -> ("error out"=w311:errorcluster, "Local Bus_Access out"=w310:refnum<class "Local Bus_CDBL.lvclass">)  [unwired: 7 in]
                          n162 = call-dynamic "Set DVR.vi"("error in (no error)"=w311, "Type Counts"=w307, "Local Bus_DBL in"=w310) -> ("error out"=w314:errorcluster, "Local Bus_DBL out"=w313:refnum<class "Local Bus_CDBL.lvclass">)  [unwired: 7 in]
                        }
                        frame "Extended Complex" {
                          n163 = Unbundle By Name(w320) -> ("CEXT"=w321:refnum<data-value>)
                          n164 = in-place {
                            in-place-border: [w329] -> w319
                            n165 = in-place-dvr #27(w321) -> (w330:cxt[])  [unwired: 1 out]
                            n166 = Array Size(array=w330) -> (size(s)=w329:i32)
                            n167 = Build Array (concatenate)(w330, cxt 0.0+0.0i ("element")) -> (w331:cxt[])
                            n168 = in-place-dvr #27(w331) -> ()  [unwired: 2 out]
                          }
                          n169 = call-dynamic "Write Index.vi"("error in (no error)"=w325, "Index"=w319, "Local Bus_Access in"=refnum<class "Local Bus_CEXT.lvclass"> refnum ("Local Bus_CEXT.lvclass")) -> ("error out"=w324:errorcluster, "Local Bus_Access out"=w323:refnum<class "Local Bus_CEXT.lvclass">)  [unwired: 7 in]
                          n170 = call-dynamic "Set DVR.vi"("error in (no error)"=w324, "Type Counts"=w320, "Local Bus_DBL in"=w323) -> ("error out"=w327:errorcluster, "Local Bus_DBL out"=w326:refnum<class "Local Bus_CEXT.lvclass">)  [unwired: 7 in]
                        }
                        frame "LabVIEW Class Instance" {
                          n171 = Unbundle By Name(w339) -> ("Type"=w340:refnum<data-value>)
                          n172 = in-place {
                            in-place-border: [w345] -> w338
                            n173 = in-place-dvr #28(w340) -> (w346:refnum<class "Abs_Type.lvclass">[])  [unwired: 1 out]
                            n174 = Array Size(array=w346) -> (size(s)=w345:i32)
                            n175 = Build Array (concatenate)(w346, refnum<class "Abs_Type.lvclass"> refnum ("element")) -> (w347:refnum<class "Abs_Type.lvclass">[])
                            n176 = in-place-dvr #28(w347) -> ()  [unwired: 2 out]
                          }
                          n177 = call-dynamic "Write Index.vi"("error in (no error)"=w343, "Index"=w338, "Local Bus_Access in"=refnum<class "Local Bus_Type.lvclass"> refnum ("Local Bus_Type.lvclass")) -> ("error out"=w342:errorcluster, "Local Bus_Access out"=w341:refnum<class "Local Bus_Type.lvclass">)  [unwired: 7 in]
                          n178 = call-dynamic "Set DVR.vi"("error in (no error)"=w342, "Type Counts"=w339, "Local Bus_DBL in"=w341) -> ("error out"=w335:errorcluster, "Local Bus_DBL out"=w334:refnum<class "Local Bus_Type.lvclass">)  [unwired: 7 in]
                          n179 = To More Specific Class(target class=refnum<class "Abs_Value.lvclass"> refnum ("Value"), reference=w334, error in=w335) -> (specific class reference=w332:refnum<class "Abs_Value.lvclass">, error out=w336:errorcluster)
                        }
                      }
                      n180 = Insert Into Map(map in=w82, key=w80, value=w75) -> (map out=w81:T4)  [unwired: 2 out]
                    }
                    frame True {
                      # "Nee to put an error here"
                    }
                  }
                }
                frame False {
                }
              }
              n181 = Bundle By Name(cluster=w54, "Tags"=w62) -> (w58:T3)
              n182 = in-place-array #7(w58) -> (w48:T3[])  [unwired: 1 out]
              n183 = in-place-match #8(w64) -> (w46:errorcluster)
            }
            n184 = in-place-cluster #5("Data"=w48) -> (w38:T2)
            n185 = in-place-match #6(w46) -> (w36:errorcluster)
          }
          n186 = in-place-dvr #3(w38) -> (w26:refnum<data-value>, w24:errorcluster)
          n187 = in-place-match #4(w36) -> (w27:errorcluster)
        }
        n188 = Merge Errors(w24, w27) -> (w25:errorcluster)
        n189 = in-place-cluster #1("Groups"=w26) -> (w18:refnum<class "Blackboard.lvclass">)
        n190 = in-place-match #2(w25) -> (w15:errorcluster)
      }
    }
    frame Error {
    }
  }
  "error out" <- w9
  "bt_Blackboard out" <- w7
  "New Tag?" <- w4
  "Value" <- w2
